vi "Own20261012_GetLoopTunnelConditionTerminal.vi"() -> ()   [LabVIEW 2024]
panel:
  out "error out":errorcluster caption="错误输出"
  out "condition_terminal_id":refnum<vi>
  in  "tunnel_id":u32
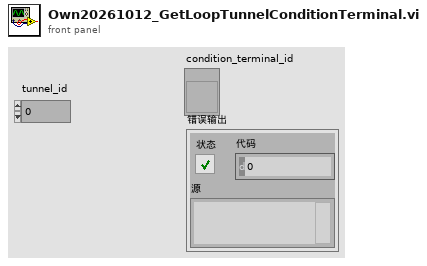
[diagram p1: front panel]
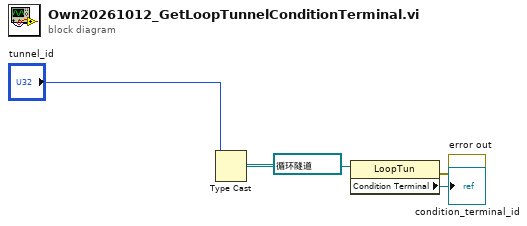
[diagram p0: block diagram]
diagram:
  n1 = Type Cast(type=refnum<vi> refnum ("引用"), x="tunnel_id") -> (*(type *) &x=w3:refnum<vi>)
  n2 = property class="LoopTun"(reference=w3) -> (error out=→"error out":errorcluster, "Condition Terminal"=→"condition_terminal_id":refnum<vi>)  [unwired: 1 in, 1 out]
